vi "INI.Attributes to Variant.vi"(8 "error in (no error)":errorcluster, 9 "Section Attribute":variant, 10 "Data Name":string, 11 "Datatype":variant) -> (0 "error out":errorcluster, 3 "Variant":variant)   [LabVIEW 2013, in "OpenSerializer.lvlib" / "Serializer.PlainText.INI.lvclass"]
doc: "JKI SMO Configuration 1.2.1.18\nJKI - JKI\nCopyright (c) 2017, JKI"
uses:
  Serializer.PlainText.INI.lvclass
  <vilib>/LabVIEW Open Source Project/Data Manipulation/TypeDescriptor/TypeDescriptor_GetName.vi
  <vilib>/LabVIEW Open Source Project/Data Manipulation/Variant/Variant_EmptyCluster.vi
  <vilib>/LabVIEW Open Source Project/Data Manipulation/TypeDescriptor/TypeDescriptor_GetPString.vi
  <vilib>/LabVIEW Open Source Project/Data Manipulation/TypeDescriptor/TypeDescriptor_SetName.vi
  <vilib>/Utility/GetType.llb/TD_Create Cluster.vi
  <vilib>/Utility/GetType.llb/TD_Get Array Information.vi
  <vilib>/Utility/GetType.llb/Get Type Code from I16 Array And Pos.vi
  <vilib>/LabVIEW Open Source Project/Data Manipulation/Conversions/Flattened nD-Array to Flattened 1D-Array.vi
  <vilib>/regexp/Match Regular Expression.xnode
  <vilib>/Utility/VariantDataType/VariantType.lvlib
  <vilib>/LabVIEW Open Source Project/Data Manipulation/Variant/OpenVariant.lvlib
  <vilib>/LabVIEW Open Source Project/Data Manipulation/TypeDescriptor/OpenDescriptor.lvlib
  Serializer.PlainText/Serializer.PlainText.lvclass
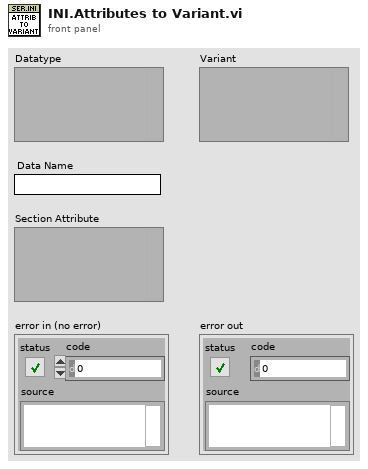
[diagram p1: front panel]
types:
  T1 = typedef "VariantType.lvlib/Type.ctl" = enum8{"Invalid Type", "Void", "I8", "I16", "I32", "I64", "U8", "U16", "U32", "U64", "Single Float", "Double Float", "Extended Float", "Single Complex", "Double Complex", "Extended Complex", "Enum U8", "Enum U16", "Enum U32", "Enum U64", "Single Float With Unit", "Double Float With Unit", "Extended Float With Unit", "Single Complex with Unit", "Double Complex with Unit", "Extended Complex with Unit", "Boolean", "String", "Path", "Picture", "Tag", "Array", "Cluster", "Variant", "LV Variant", "Waveform", "Timestamp", "Digital Waveform", "Digital Data", "ExpressData", "Refnum", "External Data", "VI", "Poly VI", "LabVIEW Class Instance", "Fixed Point"}
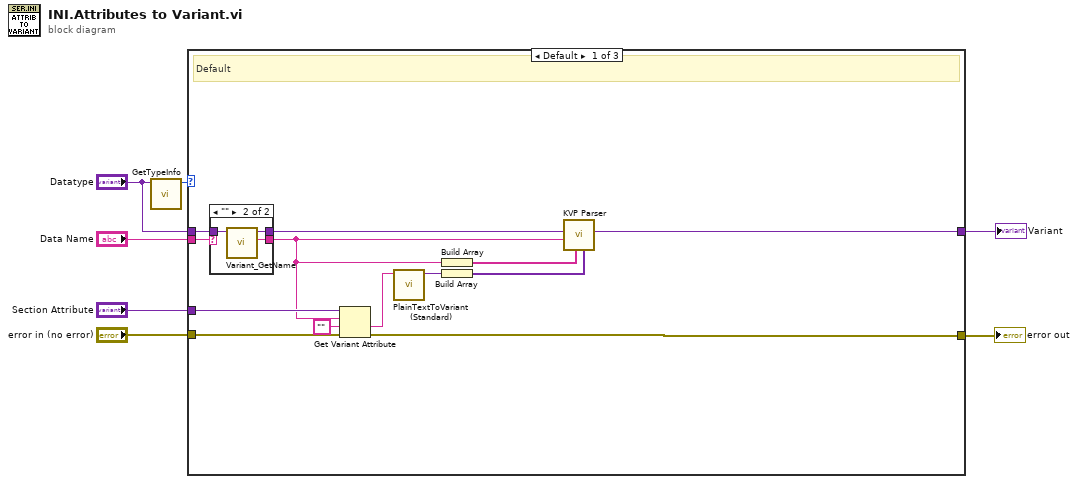
[diagram p0: block diagram]
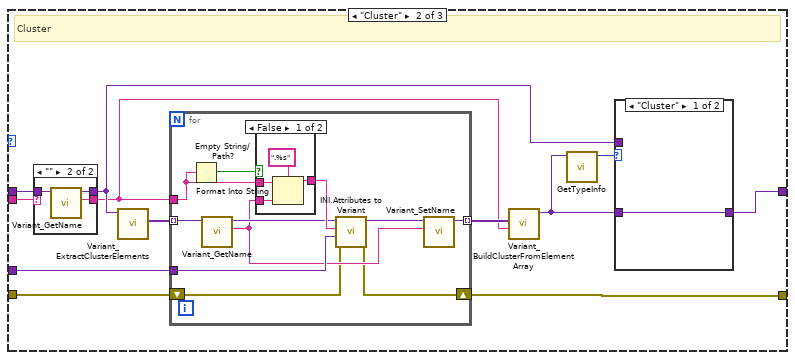
[diagram p3: hidden frame]
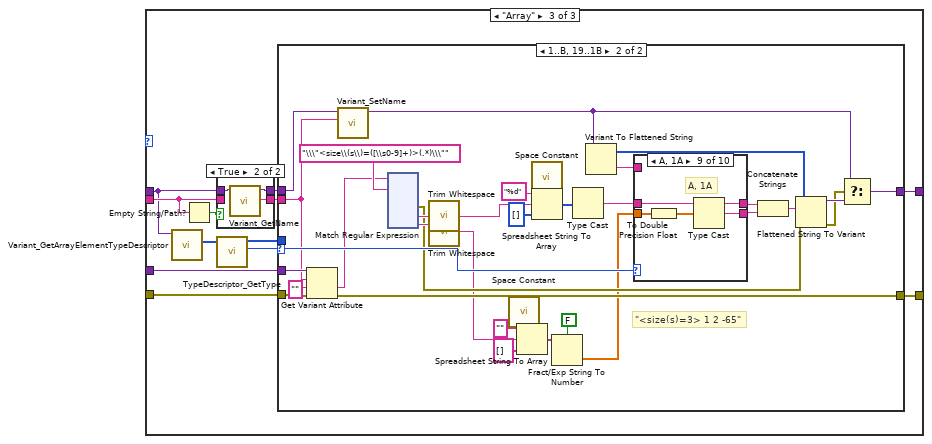
[diagram p7: hidden frame]
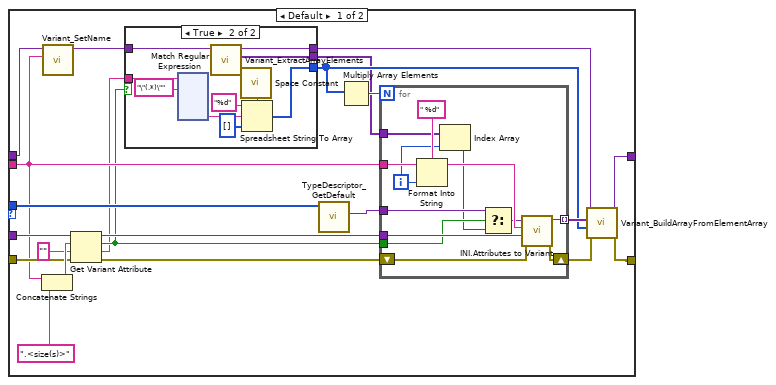
[diagram p9: hidden frame]
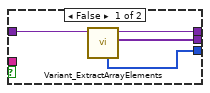
[diagram p10: hidden frame]
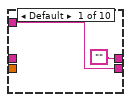
[diagram p11: hidden frame]
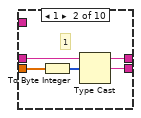
[diagram p12: hidden frame]
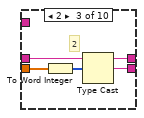
[diagram p13: hidden frame]
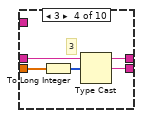
[diagram p14: hidden frame]
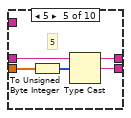
[diagram p15: hidden frame]
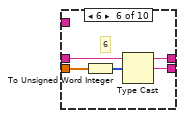
[diagram p16: hidden frame]
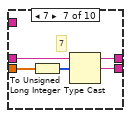
[diagram p17: hidden frame]
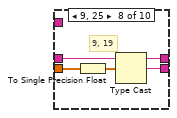
[diagram p18: hidden frame]
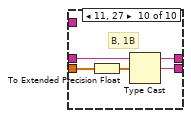
[diagram p19: hidden frame]
diagram:
  n1 = call <vilib>:"GetTypeInfo.vi"("Variant"="Datatype") -> ("Type Enum"=w1:T1)  [unwired: 6 in, 4 out]
  n2 = case shown="Default" w1 {
    tunnel: [w10 w36 w71] -> w3
    tunnel: [w19 w32 w70] -> w4
    tunnel: "Data Name" -> [w17 w26 w66]
    tunnel: "Datatype" -> [w18 w29 w64]
    tunnel: "Section Attribute" -> [w20 w37 w72]
    tunnel: "error in (no error)" -> [w12 w30 w65]
    frame Default {
      # "Default"
      n3 = case shown="\"\"" w17 {
        selector: w17 -> [w21 _]
        tunnel: w18 -> [w22 w24]
        tunnel: [w22 w23] -> w14
        tunnel: [w21 w25] -> w11
        frame Default {
        }
        frame "" {
          n4 = call <vilib>:"Variant_GetName.vi"("Variant"=w24) -> ("Name"=w25:string, "Variant dup"=w23:variant)  [unwired: 8 in, 1 out]
        }
      }
      n5 = Get Variant Attribute(Variant=w20, name=w11, default value (empty Variant)="", error in=w12) -> (value=w9:string, error out=w19:errorcluster)  [unwired: 2 out]
      n6 = call "PlainTextToVariant (Standard).vi"("String-formatted Value"=w9) -> ("Variant-formatted Value"=w8:variant)  [unwired: 9 in, 1 out]
      n7 = Build Array(w11) -> (w15:string[])
      n8 = Build Array(w8) -> (w16:variant[])
      n9 = call <vilib>:"KVP Parser.vi"("Values"=w16, "Keys"=w15, "Default Value Name (empty: label)"=w11, "Default Value"=w14) -> ("Value"=w10:variant)  [unwired: 4 in, 3 out]
    }
    frame "Cluster" {
      # "Cluster"
      n10 = case shown="\"\"" w26 {
        selector: w26 -> [w38 _]
        tunnel: w29 -> [w39 w41]
        tunnel: [w39 w40] -> w28
        tunnel: [w38 w42] -> w27
        frame Default {
        }
        frame "" {
          n11 = call <vilib>:"Variant_GetName.vi"("Variant"=w41) -> ("Name"=w42:string, "Variant dup"=w40:variant)  [unwired: 8 in, 1 out]
        }
      }
      n12 = call <vilib>:"Variant_ExtractClusterElements.vi"("Cluster"=w28) -> ("Elements"=w31:variant[])  [unwired: 8 in, 2 out]
      n13 = for {
        tunnel: w31 -> [w49] mode=indexing
        shift-right: [w45] -> w32
        shift-left: w30 -> [w46]
        tunnel: w27 -> [w53]
        tunnel: [w50] -> w34 mode=indexing
        tunnel: w37 -> [w54]
        n14 = Empty String/Path?(string/path=w53) -> (empty?=w52:bool)
        n15 = call <vilib>:"Variant_GetName.vi"("Variant"=w49) -> ("Name"=w47:string, "Variant dup"=w48:variant)  [unwired: 8 in, 1 out]
        n16 = case shown="False" w52 {
          tunnel: w47 -> [w58 w60]
          tunnel: [w57 w60] -> w55
          tunnel: w53 -> [w56 _]
          frame False {
            n17 = Format Into String(format string=".%s" ("Format String"), initial string=w56, w58) -> (resulting string=w57:string)  [unwired: 1 in, 1 out]
          }
          frame True {
          }
        }
        n18 = call "INI.Attributes to Variant.vi"("error in (no error)"=w46, "Section Attribute"=w54, "Data Name"=w55, "Datatype"=w48) -> ("error out"=w45:errorcluster, "Variant"=w51:variant)  [unwired: 6 in]
        n19 = call <vilib>:"Variant_SetName.vi"("Name"=w47, "Variant"=w51) -> ("Named Variant"=w50:variant)  [unwired: 9 in]
      }
      n20 = call <vilib>:"Variant_BuildClusterFromElementArray.vi"("name"=w27, "Elements"=w34) -> ("Cluster"=w33:variant)  [unwired: 9 in]
      n21 = call <vilib>:"GetTypeInfo.vi"("Variant"=w33) -> ("Type Enum"=w35:T1)  [unwired: 6 in, 4 out]
      n22 = case shown="\"Cluster\"" w35 {
        tunnel: w28 -> [_ w44]
        tunnel: [w43 w44] -> w36
        tunnel: w33 -> [w43 _]
        frame "Cluster" {
        }
        frame Default {
        }
      }
    }
    frame "Array" {
      n23 = call <vilib>:"Variant_GetArrayElementTypeDescriptor.vi"("Array"=w64) -> ("Element Descriptor"=w63:i16[])  [unwired: 8 in, 2 out]
      n24 = Empty String/Path?(string/path=w66) -> (empty?=w69:bool)
      n25 = case shown="True" w69 {
        tunnel: w64 -> [w73 w77]
        tunnel: [w73 w76] -> w68
        tunnel: [w74 w75] -> w67
        tunnel: w66 -> [w74 _]
        frame False {
        }
        frame True {
          n26 = call <vilib>:"Variant_GetName.vi"("Variant"=w77) -> ("Name"=w75:string, "Variant dup"=w76:variant)  [unwired: 8 in, 1 out]
        }
      }
      n27 = call <vilib>:"TypeDescriptor_GetType.vi"("type descriptor"=w63) -> ("Type"=w61:u8, "type descriptor dup"=w62:i16[])  [unwired: 9 in]
      n28 = case shown="1..B, 19..1B" w61 {
        selector: w61 -> [_ w264]
        tunnel: w68 -> [w81 w250]
        tunnel: [w88 w265] -> w71
        tunnel: [w86 w254] -> w70
        tunnel: w72 -> [w97 w275]
        tunnel: w65 -> [w91 w273]
        tunnel: w67 -> [w85 w251]
        tunnel: w62 -> [w90 _]
        frame Default {
          n29 = Concatenate Strings(w85, ".<size(s)>" ("Substring")) -> (w96:string)
          n30 = call <vilib>:"Variant_SetName.vi"("Name"=w85, "Variant"=w81) -> ("Named Variant"=w79:variant)  [unwired: 9 in]
          n31 = Get Variant Attribute(Variant=w97, name=w96, default value (empty Variant)="" ("Substring")) -> (duplicate Variant=w93:variant, found=w84:bool, value=w83:string)  [unwired: 1 in, 1 out]
          n32 = case shown="True" w84 {
            tunnel: w83 -> [_ w111]
            tunnel: [w99 w106] -> w82
            tunnel: w79 -> [w102 w105]
            tunnel: [w101 w104] -> w80
            tunnel: [w100 w103] -> w78
            frame False {
              n33 = call <vilib>:"Variant_ExtractArrayElements.vi"("Array"=w102) -> ("Elements"=w101:variant[], "Array dup"=w100:variant, "Dimensions"=w99:u32[])  [unwired: 7 in, 1 out]
            }
            frame True {
              n34 = xnode "Match Regular Expression"("input string"=w111, "regular expression"="\"(.*)\"") -> ("submatch 1"=w107:string)  [unwired: 4 in, 5 out]
              n35 = call <vilib>:"Variant_ExtractArrayElements.vi"("Array"=w105) -> ("Elements"=w104:variant[], "Array dup"=w103:variant)  [unwired: 7 in, 2 out]
              n36 = call <vilib>:"Space Constant.vi"() -> ("String"=w110:string)
              n37 = Spreadsheet String To Array(delimiter (Tab)=w110, format string="%d", spreadsheet string=w107, array type (2D Dbl)=u32[] [] ("Array Constant")) -> (array=w106:u32[])
            }
          }
          n38 = call <vilib>:"TypeDescriptor_GetDefault.vi"("type descriptor"=w90) -> ("Default"=w92:variant)  [unwired: 8 in, 2 out]
          n39 = Multiply Array Elements(1:w82) -> (0:w94:u32)
          n40 = for {
            N: w94 -> [_]
            tunnel: w93 -> [w241]
            tunnel: w92 -> [w233]
            tunnel: [w240] -> w89 mode=indexing
            tunnel: w85 -> [w237]
            shift-right: [w229] -> w87
            shift-left: w91 -> [w230]
            tunnel: w80 -> [w236]
            tunnel: w84 -> [w234]
            i -> [w235]
            n41 = Format Into String(format string=" %d" ("Format String"), initial string=w237, w235) -> (resulting string=w238:string)  [unwired: 1 in, 1 out]
            n42 = Index Array(array=w236, index=w235) -> (element=w232:variant)
            n43 = Select(t=w233, s=w234, f=w232) -> (s? t:f=w231:variant)
            n44 = call "INI.Attributes to Variant.vi"("error in (no error)"=w230, "Section Attribute"=w241, "Data Name"=w238, "Datatype"=w231) -> ("error out"=w229:errorcluster, "Variant"=w240:variant)  [unwired: 6 in]
          }
          n45 = call <vilib>:"Variant_BuildArrayFromElementArray.vi"("error in (no error)"=w87, "Dimensions"=w82, "Elements"=w89, "Default Array"=w78) -> ("error out"=w86:errorcluster, "Output Array"=w88:variant)  [unwired: 6 in]
        }
        frame 1..11, 25..27 {
          # "\"<size(s)=3> 1 2 -65\""
          n46 = Get Variant Attribute(Variant=w275, name=w251, default value (empty Variant)="", error in=w273) -> (value=w257:string, error out=w254:errorcluster)  [unwired: 2 out]
          n47 = call <vilib>:"Variant_SetName.vi"("Name"=w251, "Variant"=w250) -> ("Named Variant"=w249:variant)  [unwired: 9 in]
          n48 = xnode "Match Regular Expression"("input string"=w257, "regular expression"="\\\"<size\\(s\\)=([\\s0-9]+)>(.*)\\\"") -> ("error out"=w252:errorcluster, "submatch 1"=w259:string, "submatch 2"=w260:string)  [unwired: 4 in, 4 out]
          n49 = call <vilib>:"Trim Whitespace.vi"("string"=w259) -> ("trimmed string"=w256:string)  [unwired: 1 in]
          n50 = call <vilib>:"Trim Whitespace.vi"("string"=w260) -> ("trimmed string"=w243:string)  [unwired: 1 in]
          n51 = call <vilib>:"Space Constant.vi"() -> ("String"=w246:string)
          n52 = Spreadsheet String To Array(delimiter (Tab)=w246, format string="", spreadsheet string=w243, array type (2D Dbl)=string[] []) -> (array=w245:string[])
          n53 = call <vilib>:"Space Constant.vi"() -> ("String"=w253:string)
          n54 = Spreadsheet String To Array(delimiter (Tab)=w253, format string="%d", spreadsheet string=w256, array type (2D Dbl)=u32[] []) -> (array=w263:u32[])
          n55 = Fract/Exp String To Number(use system decimal point (T)=FALSE, string=w245) -> (number=w242:dbl[])  [unwired: 2 in, 1 out]
          n56 = Type Cast(x=w263) -> (*(type *) &x=w255:string)  [unwired: 1 in]
          n57 = Variant To Flattened String(Variant=w249) -> (data string=w270:string, 1:w269:i16[])
          n58 = case shown="A, 1A" w264 {
            tunnel: w242 -> [_ w398 w402 w406 w410 w414 w418 w422 w424 w428]
            tunnel: [w393 w396 w400 w404 w408 w412 w416 w420 w426 w430] -> w267
            tunnel: ["" w395 w399 w403 w407 w411 w415 w419 w425 w429] -> w268
            tunnel: w255 -> [_ w395 w399 w403 w407 w411 w415 w419 w425 w429]
            tunnel: w270 -> [w393 _ _ _ _ _ _ _ _ _]
            frame Default {
            }
            frame 1 {
              # "1"
              n59 = To Byte Integer(number=w398) -> (8bit integer=w397:i8[])
              n60 = Type Cast(x=w397) -> (*(type *) &x=w396:string)  [unwired: 1 in]
            }
            frame 2 {
              # "2"
              n61 = To Word Integer(number=w402) -> (16bit integer=w401:i16[])
              n62 = Type Cast(x=w401) -> (*(type *) &x=w400:string)  [unwired: 1 in]
            }
            frame 3 {
              # "3"
              n63 = To Long Integer(number=w406) -> (32bit integer=w405:i32[])
              n64 = Type Cast(x=w405) -> (*(type *) &x=w404:string)  [unwired: 1 in]
            }
            frame 5 {
              # "5"
              n65 = To Unsigned Byte Integer(number=w410) -> (unsigned 8bit integer=w409:u8[])
              n66 = Type Cast(x=w409) -> (*(type *) &x=w408:string)  [unwired: 1 in]
            }
            frame 6 {
              # "6"
              n67 = To Unsigned Word Integer(number=w414) -> (unsigned 16bit integer=w413:u16[])
              n68 = Type Cast(x=w413) -> (*(type *) &x=w412:string)  [unwired: 1 in]
            }
            frame 7 {
              # "7"
              n69 = To Unsigned Long Integer(number=w418) -> (unsigned 32bit integer=w417:u32[])
              n70 = Type Cast(x=w417) -> (*(type *) &x=w416:string)  [unwired: 1 in]
            }
            frame 9, 25 {
              # "9, 19"
              n71 = To Single Precision Float(number=w422) -> (single precision float=w421:sgl[])
              n72 = Type Cast(x=w421) -> (*(type *) &x=w420:string)  [unwired: 1 in]
            }
            frame 10, 26 {
              # "A, 1A"
              n73 = To Double Precision Float(number=w424) -> (double precision float=w423:dbl[])
              n74 = Type Cast(x=w423) -> (*(type *) &x=w426:string)  [unwired: 1 in]
            }
            frame 11, 27 {
              # "B, 1B"
              n75 = To Extended Precision Float(1:w428) -> (0:w427:ext[])
              n76 = Type Cast(x=w427) -> (*(type *) &x=w430:string)  [unwired: 1 in]
            }
          }
          n77 = Concatenate Strings(w268, w267) -> (w266:string)
          n78 = Flattened String To Variant(4:w252, 6:w266, 7:w269) -> (0:w271:errorcluster, 3:w272:variant)
          n79 = Select(t=w249, s=w271, f=w272) -> (s? t:f=w265:variant)
        }
      }
    }
  }
  "error out" <- w4
  "Variant" <- w3
